vi "Documentation.vi"() -> (0 "Author":string, 1 "History":string, 2 "Version":string, 3 "Description":string)   [LabVIEW 2021, in "CAN_Writer_CANsub_Plugin.lvlib"]
uses:
  CAN_Writer_CANsub_Plugin.lvlib
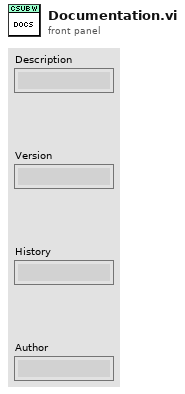
[diagram p1: front panel]
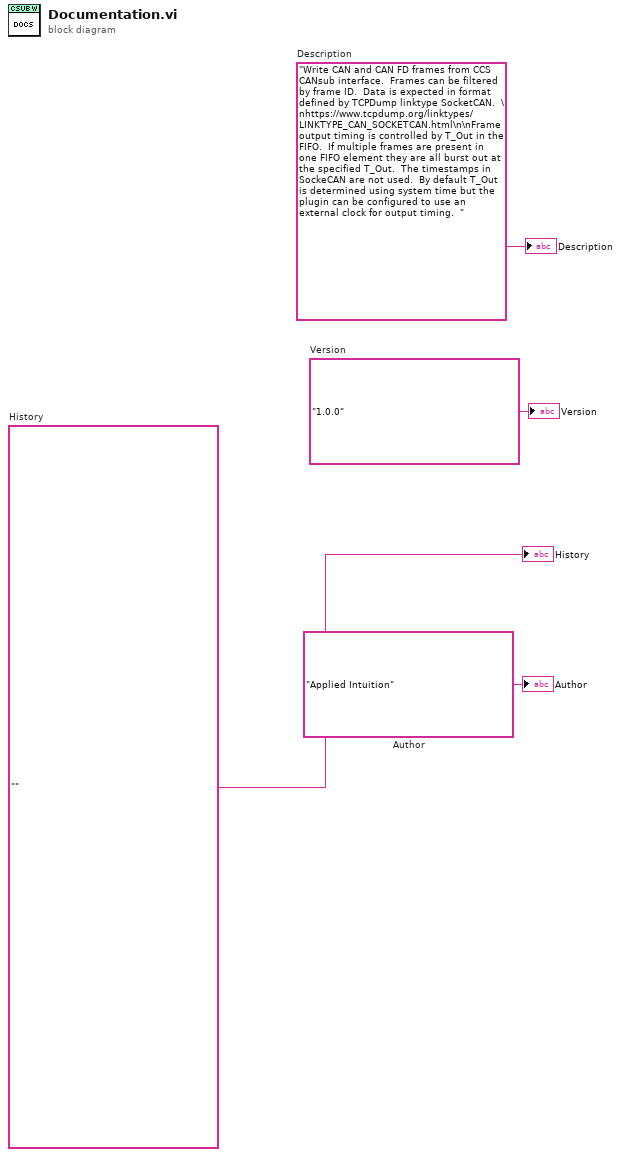
[diagram p0: block diagram]
diagram:
  w1 = "Applied Intuition"  # Author
  w2 = ""  # History
  w3 = "1.0.0"  # Version
  w4 = "Write CAN and CAN FD frames from CCS CANsub interface.  Frames can be filtered by frame ID.  Data is expected in format defined by TCPDump linktype SocketCAN.  \nhttps://www.tcpdump.org/linktypes/LINKTYPE_CAN_SOCKETCAN.html\n\nFrame output timing is controlled by T_Out in the FIFO.  If multiple frames are present in one FIFO element they are all burst out at the specified T_Out.  The timestamps in SockeCAN are not used.  By default T_Out is determined using system time but the plugin can be configured to use an external clock for output timing.  "  # Description
  "Description" <- w4
  "Version" <- w3
  "History" <- w2
  "Author" <- w1
